vi "SpO2_Manual_Processing.vi"() -> ()   [LabVIEW 2018]
uses:
  <vilib>/Analysis/3filter.llb/Filter Passband Type.ctl
  <vilib>/Analysis/1siggen.llb/Ramp Pattern by Samples.vi
  <vilib>/Utility/file.llb/Read Delimited Spreadsheet (DBL).vi
  <vilib>/Analysis/3filter.llb/Butterworth Filter (DBL).vi
  <vilib>/Utility/file.llb/Write Delimited Spreadsheet (DBL).vi
  <vilib>/Analysis/NI_AALBase.lvlib
panel:
  out "X Position (Infrared)":dbl
  out "Y Position (Infrared)":dbl
  out "Y Position (Red)":dbl
  out "X Position (Red)":dbl
  in  "Button":bool
  out "IR PPG":cluster{dbl[], dbl[]}(graph) caption="Raw PPG"
  out "Raw PPG 2":cluster{dbl[], dbl[]}(graph) caption="Raw PPG"
  in  "Interval (s)":dbl
  in  "Begin (s)":dbl
  out "Raw PPG":cluster{dbl[], dbl[]}[](graph)
  in  "Sampling Frequency(Hz)":dbl=500.0
  # "Raw PPG"
  # "Red PPG"
  # "IR PPG"
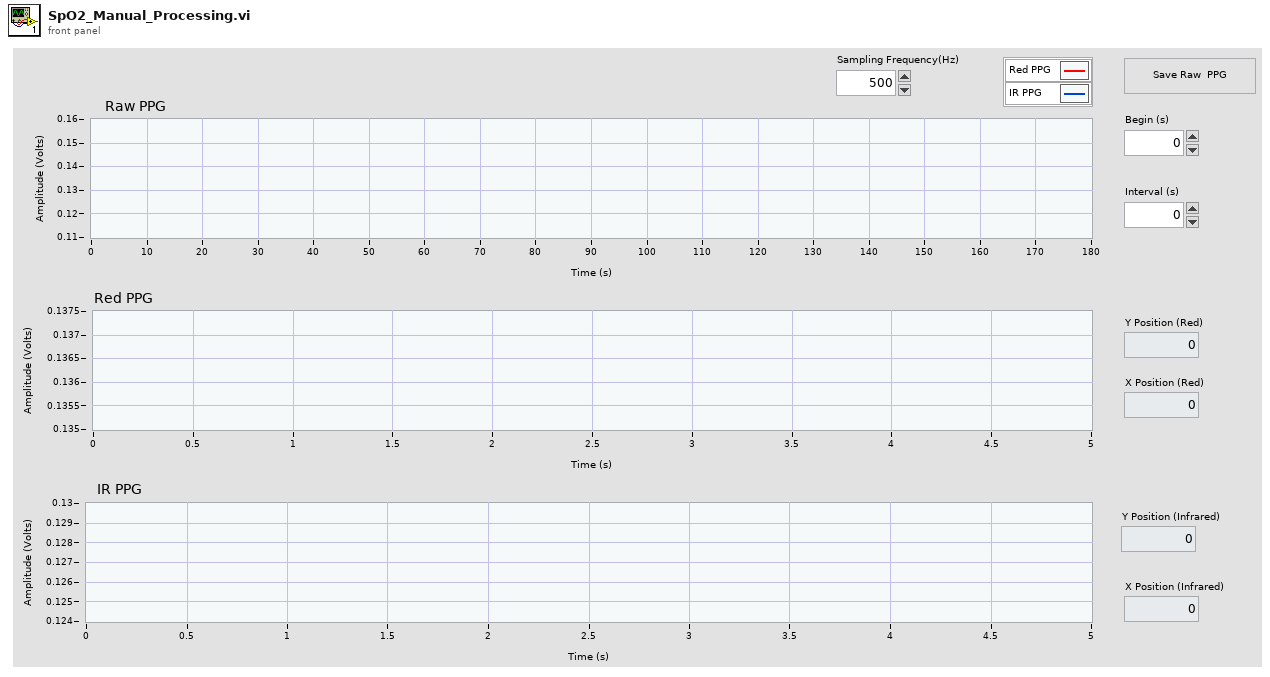
[diagram p1: front panel]
types:
  T1 = typedef "NI_AALBase.lvlib/Filter Passband Type.ctl" = enum32{"Lowpass", "Highpass", "Bandpass", "Bandstop"}
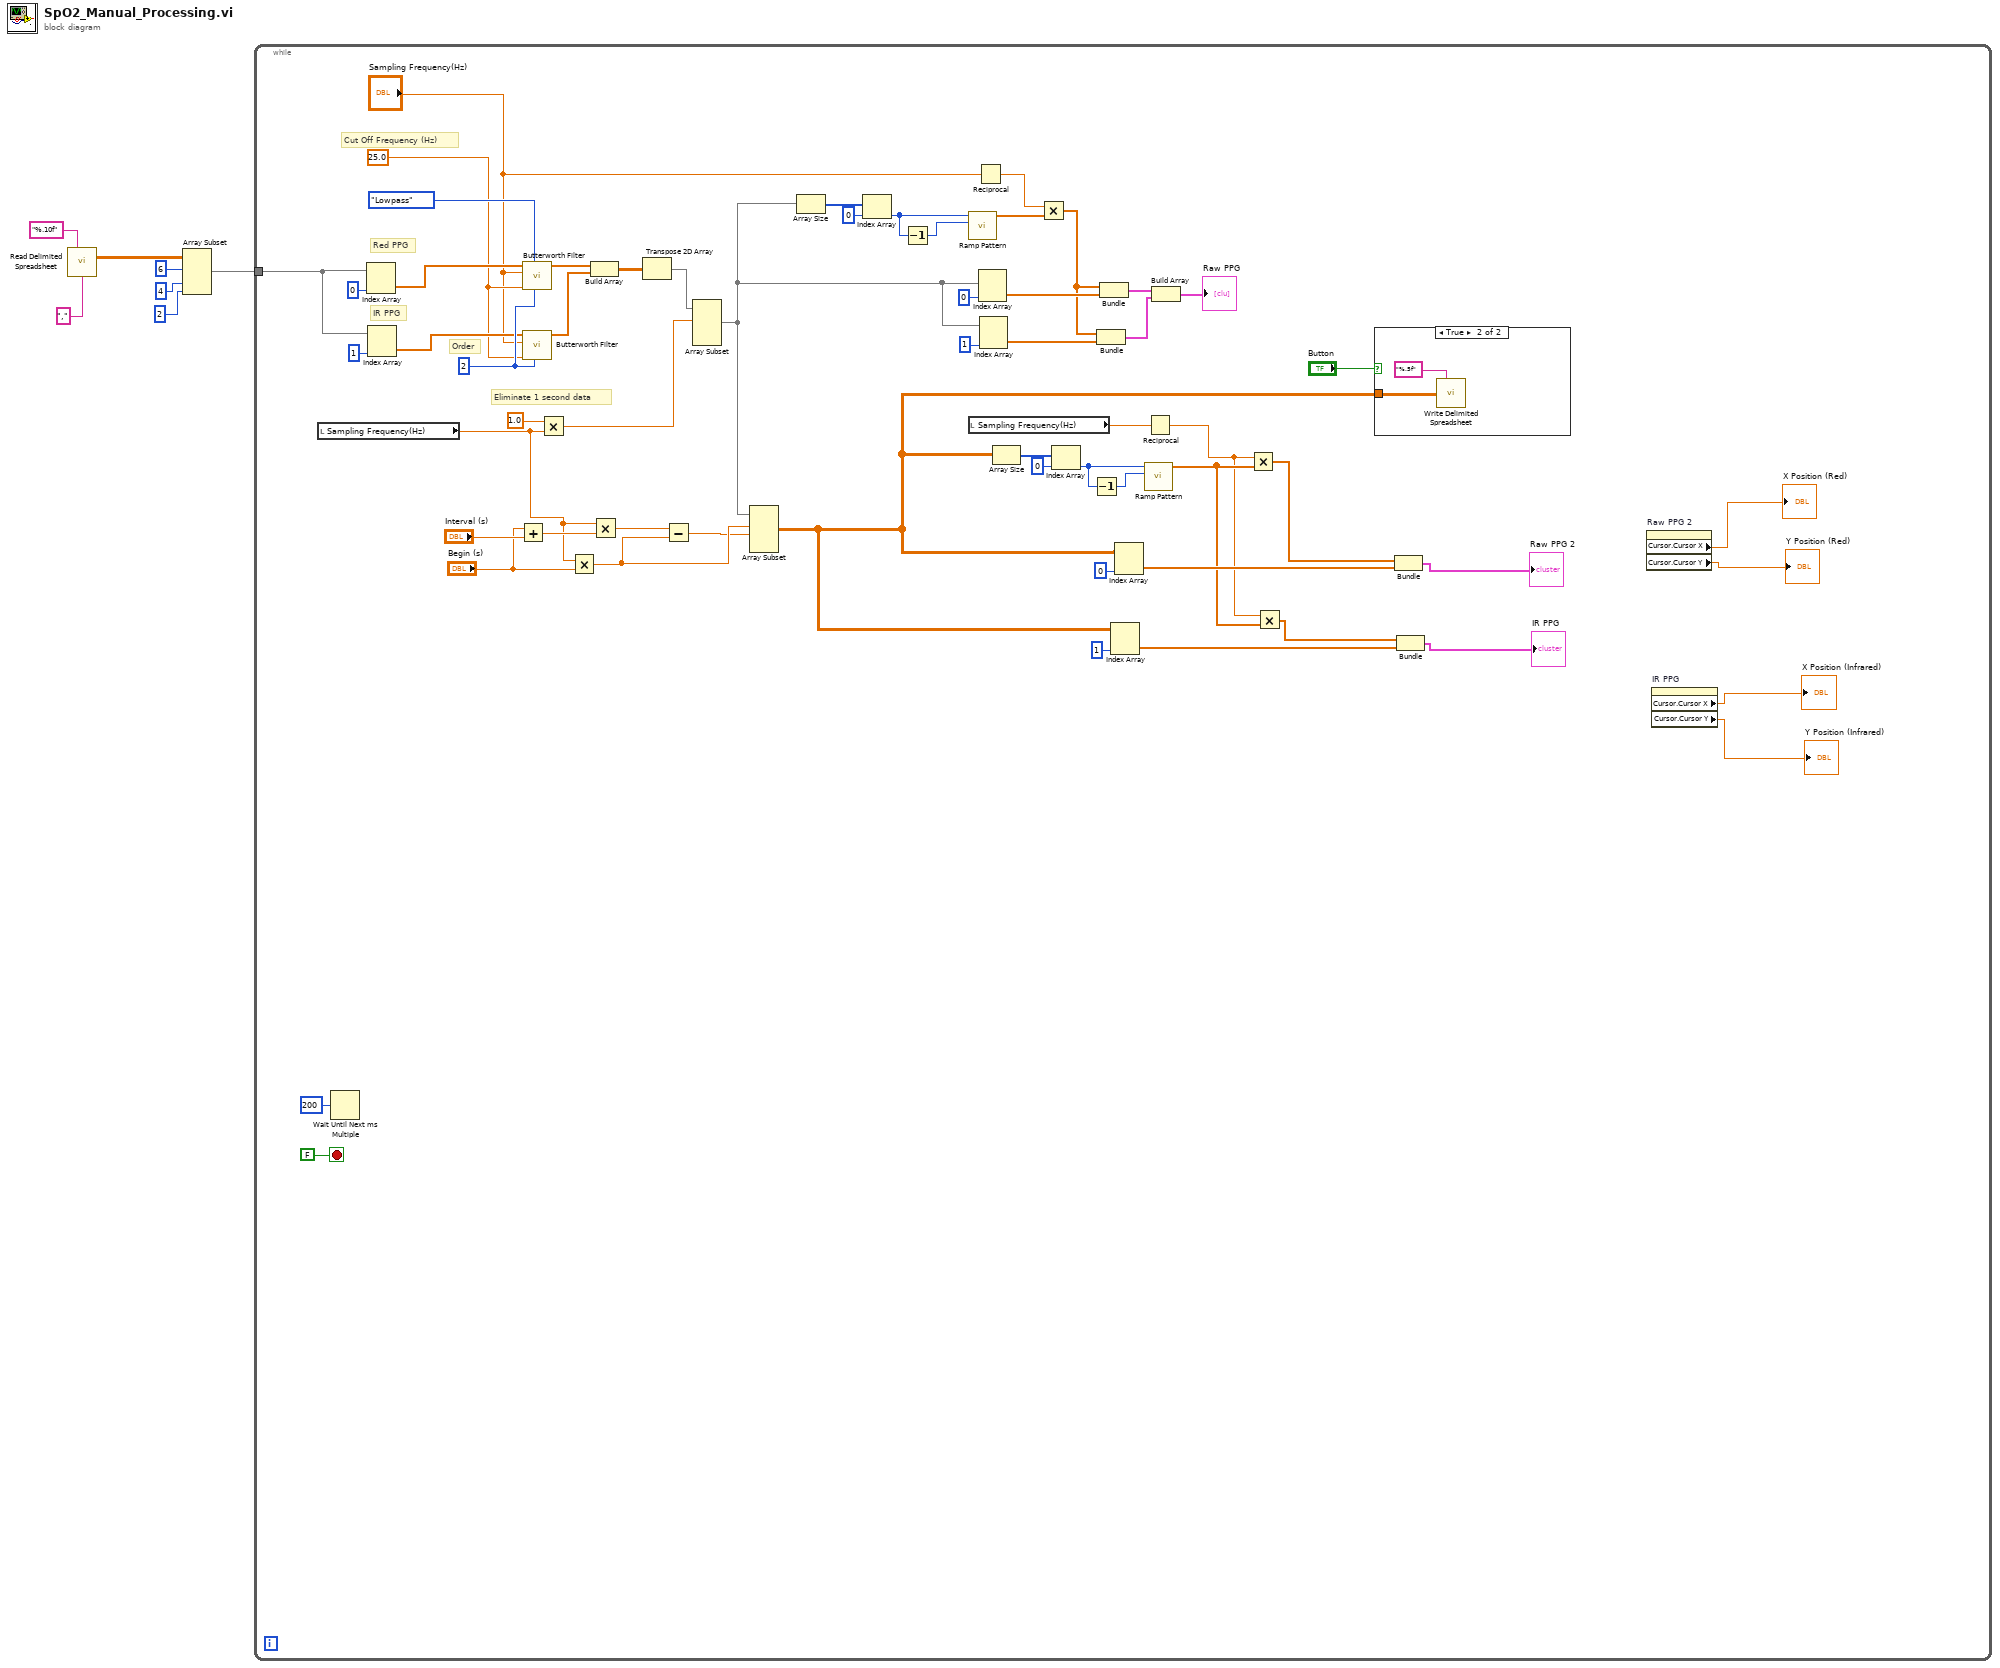
[diagram p0: block diagram]
diagram:
  n1 = call-poly <vilib>:"Read Delimited Spreadsheet.vi"("format (%.3f)"="%.10f", "delimiter (\\t)"=",") -> ("all rows"=w5:dbl[][])  [unwired: 8 in, 5 out]
  n2 = Array Subset(array=w5, index (row)=6 ("index"), index (col)=4 ("disabled index (col)"), length (col)=2 ("disabled index (col)")) -> (w1:dbl[][])  [unwired: 1 in]
  n3 = while {
    tunnel: w1 -> [w64]
    stop <- FALSE stop-if-true
    w60 = 25.0 ("Cutoff Frequency(Hz)")
    w62 = 2 ("order")
    # "Cut Off Frequency (Hz)"
    # "Eliminate 1 second data"
    # "IR PPG"
    # "Red PPG"
    # "Order"
    n4 = local read "Sampling Frequency(Hz)"() -> (w25:dbl)
    n5 = Wait Until Next ms Multiple(millisecond multiple=u32 200) -> ()  [unwired: 1 out]
    n6 = Index Array(array=w64, index (col)=0 ("disabled index (col)")) -> (element=w63:dbl[])  [unwired: 1 in]
    n7 = Index Array(array=w64, index (col)=1 ("disabled index (col)")) -> (element=w61:dbl[])  [unwired: 1 in]
    n8 = Add(x="Begin (s)", y="Interval (s)") -> (x+y=w28:dbl)
    n9 = call-poly <vilib>:"Butterworth Filter.vi"("order"=w62, "filter type"=Filter_Passband_Type."Lowpass", "low cutoff freq: fl"=w60, "sampling freq: fs"="Sampling Frequency(Hz)", "X"=w63) -> ("Filtered X"=w59:dbl[])  [unwired: 3 in, 1 out]
    n10 = call-poly <vilib>:"Butterworth Filter.vi"("order"=w62, "low cutoff freq: fl"=w60, "sampling freq: fs"="Sampling Frequency(Hz)", "X"=w61) -> ("Filtered X"=w58:dbl[])  [unwired: 4 in, 1 out]
    n11 = Multiply(x=1.0, y=w25) -> (x*y=w31:dbl)
    n12 = Multiply(x=w25, y="Begin (s)") -> (x*y=w38:dbl)
    n13 = Build Array(w59, w58) -> (w57:dbl[][])
    n14 = Multiply(x=w25, y=w28) -> (x*y=w39:dbl)
    n15 = Transpose 2D Array(2D array=w57) -> (transposed array=w56:dbl[][])
    n16 = Subtract(x=w39, y=w38) -> (x-y=w27:dbl)
    n17 = Array Subset(array=w56, index (row)=w31) -> (w40:dbl[][])  [unwired: 3 in]
    n18 = Array Subset(array=w40, index (row)=w38, length (row)=w27) -> (w14:dbl[][])  [unwired: 2 in]
    n19 = Array Size(array=w40) -> (size(s)=w55:i32[])
    n20 = Index Array(array=w55, index=0) -> (element=w53:i32)
    n21 = Decrement(x=w53) -> (x-1=w52:i32)
    n22 = call-poly <vilib>:"Ramp Pattern.vi"("end"=w52, "samples"=w53) -> ("Ramp Pattern"=w51:dbl[])  [unwired: 8 in, 1 out]
    n23 = local read "Sampling Frequency(Hz)"() -> (w21:dbl)
    n24 = Reciprocal(x="Sampling Frequency(Hz)") -> (1/x=w45:dbl)
    n25 = Index Array(array=w40, index (col)=0 ("disabled index (col)")) -> (element=w46:dbl[])  [unwired: 1 in]
    n26 = Index Array(array=w40, index (col)=1) -> (element=w42:dbl[])  [unwired: 1 in]
    n27 = Array Size(array=w14) -> (size(s)=w32:i32[])
    n28 = Multiply(x=w45, y=w51) -> (x*y=w44:dbl[])
    n29 = Index Array(array=w32, index=0) -> (element=w34:i32)
    n30 = Decrement(x=w34) -> (x-1=w35:i32)
    n31 = Bundle(w44, w42) -> (w41:cluster{dbl[], dbl[]})  [unwired: 1 in]
    n32 = Bundle(w44, w46) -> (w48:cluster{dbl[], dbl[]})  [unwired: 1 in]
    n33 = Index Array(array=w14, index (col)=1 ("disabled index (col)")) -> (element=w20:dbl[])  [unwired: 1 in]
    n34 = Index Array(array=w14, index (col)=0 ("disabled index (col)")) -> (element=w22:dbl[])  [unwired: 1 in]
    n35 = call-poly <vilib>:"Ramp Pattern.vi"("end"=w35, "samples"=w34) -> ("Ramp Pattern"=w17:dbl[])  [unwired: 8 in, 1 out]
    n36 = Reciprocal(x=w21) -> (1/x=w16:dbl)
    n37 = Build Array(w48, w41) -> (→"Raw PPG":cluster{dbl[], dbl[]}[])
    n38 = Multiply(x=w16, y=w17) -> (x*y=w37:dbl[])
    n39 = Multiply(x=w16, y=w17) -> (x*y=w18:dbl[])
    n40 = case shown="True" "Button" {
      tunnel: w14 -> [_ w69]
      frame False {
      }
      frame True {
        n41 = call-poly <vilib>:"Write Delimited Spreadsheet.vi"("format (%.3f)"="%.5f", "2D data"=w69) -> ()  [unwired: 12 in, 2 out]
      }
    }
    n42 = Bundle(w37, w22) -> (→"Raw PPG 2":cluster{dbl[], dbl[]})  [unwired: 1 in]
    n43 = Bundle(w18, w20) -> (→"IR PPG":cluster{dbl[], dbl[]})  [unwired: 1 in]
    n44 = property on="Raw PPG 2" class="XYGraph (strict)"() -> ("Cursor.Cursor X"=→"X Position (Red)":dbl, "Cursor.Cursor Y"=→"Y Position (Red)":dbl)  [unwired: 2 in, 2 out]
    n45 = property on="IR PPG" class="XYGraph (strict)"() -> ("Cursor.Cursor X"=→"X Position (Infrared)":dbl, "Cursor.Cursor Y"=→"Y Position (Infrared)":dbl)  [unwired: 2 in, 2 out]
  }
